vi "VIH - CHM Project - Write IDX File.vi"(8 "error in":errorcluster, 9 "Project Files":T2, 10 "Target IDX File":path, 11 "Template IDX File":path) -> (0 "error out":errorcluster)   [LabVIEW 2014]
doc: "::: VI Helpeks :::\nCopyright (c) 2000-2026 Konstantin Shifershteyn. All rights reserved."
uses:
  _VIH HelpGen - Palette.llb/VIH HelpGen Typedef - Palette - Item Type Enum.ctl
panel:
  # "VI Helpeks\nCopyright (c) 2012-2026 Konstantin Shifershteyn"
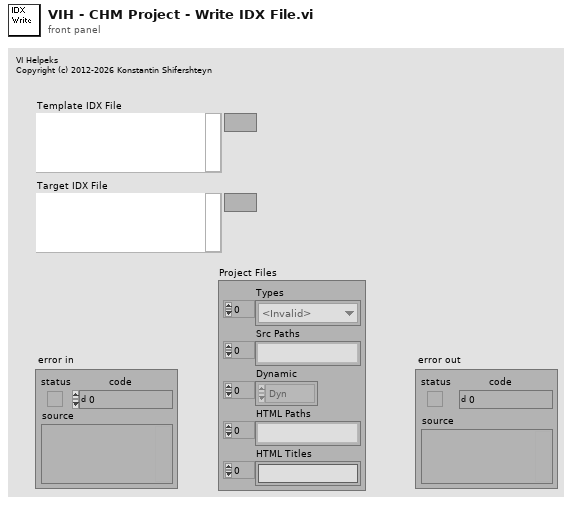
[diagram p1: front panel]
types:
  T1 = typedef "VIH HelpGen Typedef - Palette - Item Type Enum.ctl" = enum32{"<Invalid>", "<unknown>", "VI", "Menu", "LV Func", "Express VI", "Poly VI", "CTL", "HTML"}
  T2 = cluster{"Types":T1[], "Src Paths":path[], "Dynamic":enum16{"Dyn", "Stat", "Both"}[], "HTML Paths":path[], "HTML Titles":string[]}
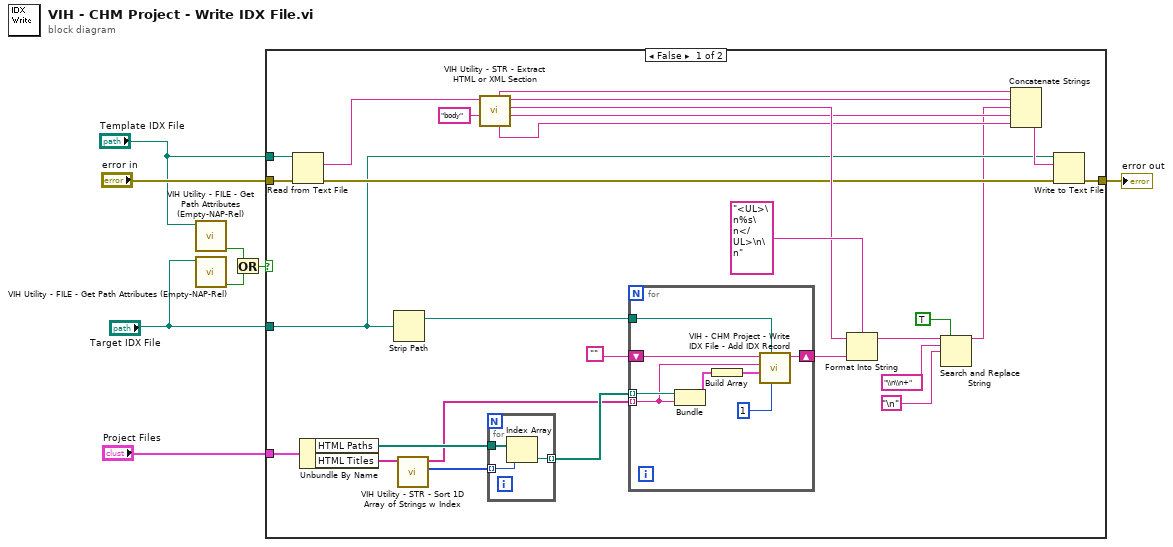
[diagram p0: block diagram]
diagram:
  n1 = call "VIH Utility - FILE - Get Path Attributes (Empty-NAP-Rel).vi"("Path"="Template IDX File") -> ("Not A Path or Empty path"=w5:bool)  [unwired: 6 in, 4 out]
  n2 = call "VIH Utility - FILE - Get Path Attributes (Empty-NAP-Rel).vi"("Path"="Target IDX File") -> ("Not A Path or Empty path"=w4:bool)  [unwired: 6 in, 4 out]
  n3 = Or(x=w5, y=w4) -> (x .or. y?=w1:bool)
  n4 = case shown="False" w1 {
    tunnel: "Template IDX File" -> [w35 _]
    tunnel: "error in" -> [w34 w48]
    tunnel: [w25 w48] -> w7
    tunnel: "Target IDX File" -> [w24 _]
    tunnel: "Project Files" -> [w19 _]
    frame False {
      n5 = Read from Text File(file (use dialog)=w35, error in=w34) -> (text=w33:string, error out=w27:errorcluster)  [unwired: 2 in, 2 out]
      n6 = Unbundle By Name(w19) -> ("HTML Paths"=w20:path[], "HTML Titles"=w22:string[])
      n7 = Strip Path(path=w24) -> (stripped path=w17:path)  [unwired: 1 out]
      n8 = call "VIH Utility - STR - Sort 1D Array of Strings w Index.vi"("Array in"=w22) -> ("Index array"=w21:i32[], "Array out"=w14:string[])  [unwired: 7 in, 2 out]
      n9 = call "VIH Utility - STR - Extract HTML or XML Section.vi"("Section name"="body", "HTML in"=w33) -> ("end"=w28:string, "body"=w31:string, "start"=w29:string, "after"=w23:string, "before"=w30:string)  [unwired: 5 in]
      n10 = for {
        tunnel: w21 -> [w47] mode=indexing
        tunnel: w20 -> [w46]
        tunnel: [w45] -> w15 mode=indexing
        n11 = Index Array(array=w46, index=w47) -> (element=w45:path)
      }
      n12 = for {
        shift-right: [w41] -> w16
        shift-left: "" -> [w43]
        tunnel: w17 -> [w42]
        tunnel: w15 -> [w44] mode=indexing
        tunnel: w14 -> [w37] mode=indexing
        n13 = Bundle(w44, "String"=w37) -> (w39:cluster{path, "String":string})  [unwired: 1 in]
        n14 = Build Array(w39) -> (w38:cluster{path, "String":string}[])
        n15 = call "VIH - CHM Project - Write IDX File - Add IDX Record.vi"("Level"=1, "Base Dir Path"=w42, "Topics"=w38, "Keyword"=w37, "HTML in"=w43) -> ("HTML out"=w41:string)  [unwired: 6 in]
      }
      n16 = Format Into String(format string="<UL>\n%s\n</UL>\n\n", initial string=w31, w16) -> (resulting string=w10:string)  [unwired: 1 in, 1 out]
      n17 = Search and Replace String(replace all?=TRUE, input string=w10, search string="\\n\\n+", replace string="\n") -> (result string=w9:string)  [unwired: 4 in, 3 out]
      n18 = Concatenate Strings(w30, w29, w9, w28, w23) -> (w26:string)
      n19 = Write to Text File(file (use dialog)=w24, text=w26, error in=w27) -> (error out=w25:errorcluster)  [unwired: 1 in, 2 out]
    }
    frame True {
    }
  }
  "error out" <- w7
